vi "RDV-sortKeysAlphabetically.vi"(8 "error in (no error)":errorcluster, 11 "RDV-Reflection_Data_viewer in":refnum<class "RDV-Reflection_Data_viewer.lvclass">) -> (0 "error out":errorcluster, 2 "Data Keys sorted":string[](array[string]), 3 "RDV-Reflection_Data_viewer out":refnum<class "RDV-Reflection_Data_viewer.lvclass">)   [LabVIEW 2020, in "RDV-Reflection_Data_viewer.lvclass"]
doc: "Sorts the keys of the viewer's data alphabetically and returns them."
uses:
  RDV-Reflection_Data_viewer.lvclass
  RDV-Reflection_Data_viewer.lvclass/RDV-Reflection_Data_viewer.ctl
  1bc6baab-a834-4652-b74b-bc8157ec794b.vi
  d423103e-ebfa-431b-8272-c8059533d061.vi
  <vilib>/Comparison/Less/Less Functor/Less Functor.lvclass
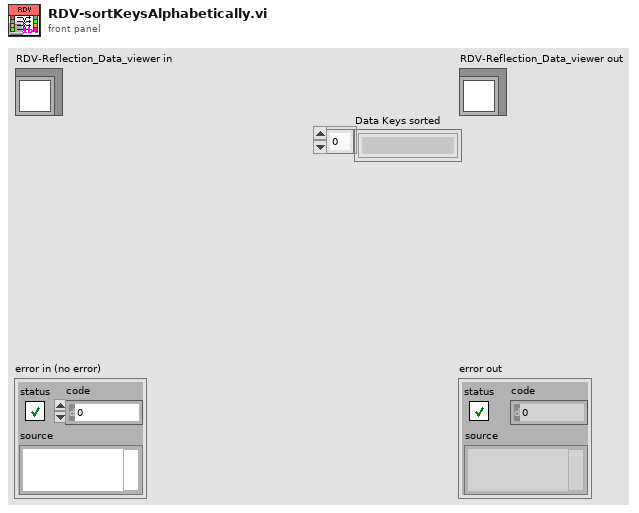
[diagram p1: front panel]
types:
  T1 = typedef "RDV-Reflection_Data_viewer.lvclass/RDV-DATA_MAP.ctl" = map{string, T2}
  T2 = typedef "RDV-Reflection_Data_viewer.lvclass/RDV-DATA_MAP_CLUST.ctl" = cluster{"filename w/ ext":string, "Common Format":T3}
  T3 = typedef "RFH-Reflection_File_Handler.lvlib/RFH-common_data_format.ctl" = cluster{"Frequency":dbl[], "Reflection'":dbl[], "Reflection''":dbl[], "Permativity'":dbl[], "Permativity''":dbl[], "Conductivity":dbl[], "Loss Tangent":dbl[], "Resistance":dbl[], "Reactance":dbl[]}
  T4 = typedef "RDV-Reflection_Data_viewer.lvclass/RDV-UPDATE_IGNORE_LIST.ctl" = string[]
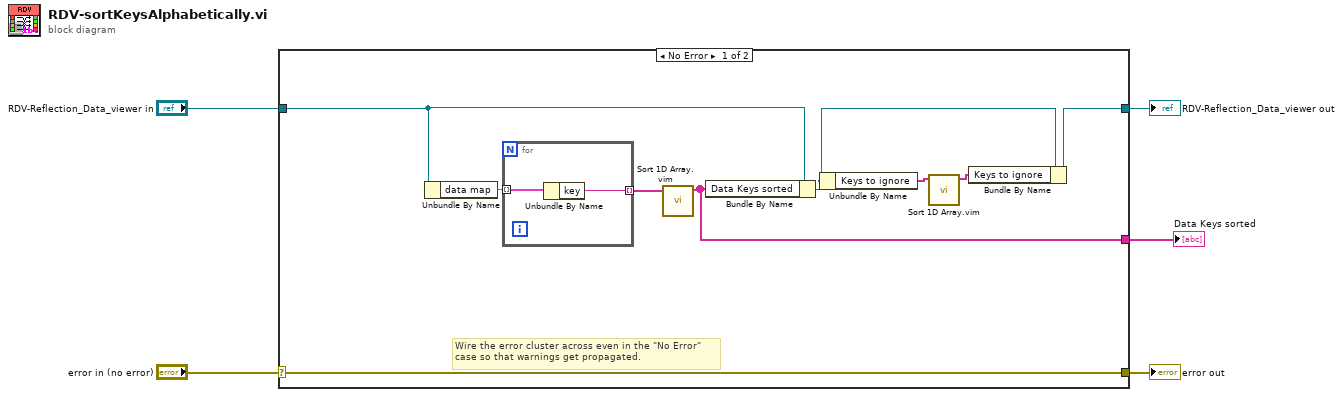
[diagram p0: block diagram]
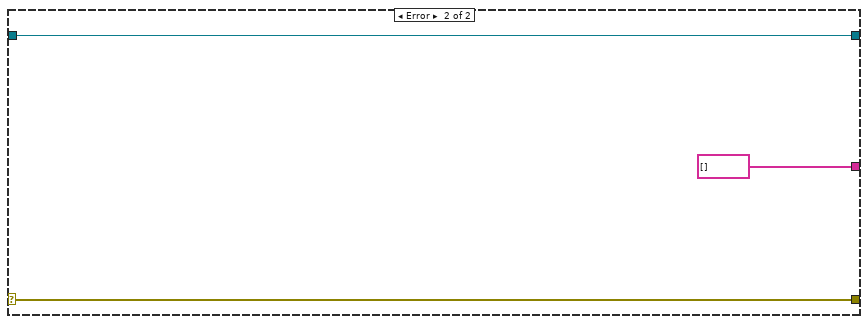
[diagram p2: hidden frame]
diagram:
  n1 = case shown="No Error" "error in (no error)" {
    selector: "error in (no error)" -> [w14 w19]
    tunnel: [w14 w19] -> w4
    tunnel: [w7 w18] -> w2
    tunnel: "RDV-Reflection_Data_viewer in" -> [w13 w18]
    tunnel: [w10 string[] [] ("sorted array")] -> w1
    frame No Error {
      # "Wire the error cluster across even in the \"No Error\"\ncase so that warnings get propagated."
      n2 = Unbundle By Name(w13) -> ("data map"=w12:T1)
      n3 = for {
        tunnel: w12 -> [w16] mode=indexing
        tunnel: [w15] -> w11 mode=indexing
        n4 = Unbundle By Name(w16) -> ("key"=w15:string)
      }
      n5 = call "Sort 1D Array.vim"("unsorted array"=w11) -> ("sorted array"=w10:string[])  [unwired: 10 in]
      n6 = Bundle By Name(cluster=w13, "Data Keys sorted"=w10) -> (w9:refnum<class "RDV-Reflection_Data_viewer.lvclass">)
      n7 = Unbundle By Name(w9) -> ("Keys to ignore"=w8:T4)
      n8 = call "Sort 1D Array.vim"("unsorted array"=w8) -> ("sorted array"=w6:T4)  [unwired: 10 in]
      n9 = Bundle By Name(cluster=w9, "Keys to ignore"=w6) -> (w7:refnum<class "RDV-Reflection_Data_viewer.lvclass">)
    }
    frame Error {
    }
  }
  "error out" <- w4
  "RDV-Reflection_Data_viewer out" <- w2
  "Data Keys sorted" <- w1
